vi "letterbox_resize_cubic_planar.vi"(7 "pad Color":u32(colorbox)=7500402, 8 "error in (no error)":errorcluster, 9 "target_h":i32=1024, 10 "target_w":i32=1024, 11 "image in":T1) -> (0 "error out":errorcluster, 1 "out_top":i32, 2 "out_left":i32, 3 "image out":T1, 4 "out_scale":sgl)   [LabVIEW 2017, in "Image Processing Library.lvlib"]
uses:
  Image Processing Library.lvlib
  <vilib>/picture/picture.llb/imagedata.ctl
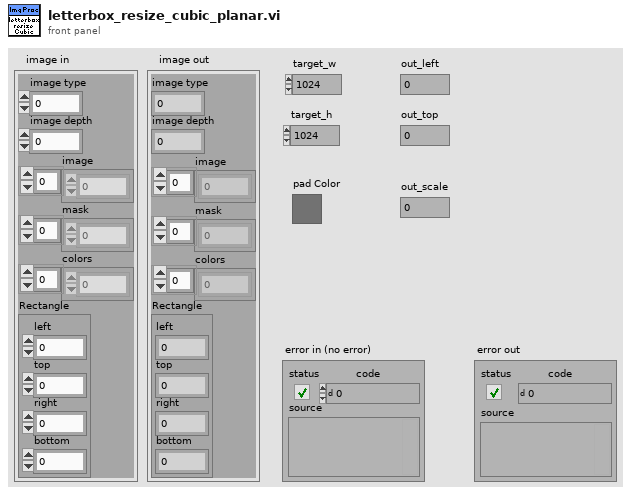
[diagram p1: front panel]
types:
  T1 = typedef "imagedata.ctl" = cluster{"image type":i32, "image depth":i32, "image":u8[], "mask":u8[], "colors":u32[], "Rectangle":cluster{"left":i16, "top":i16, "right":i16, "bottom":i16}}
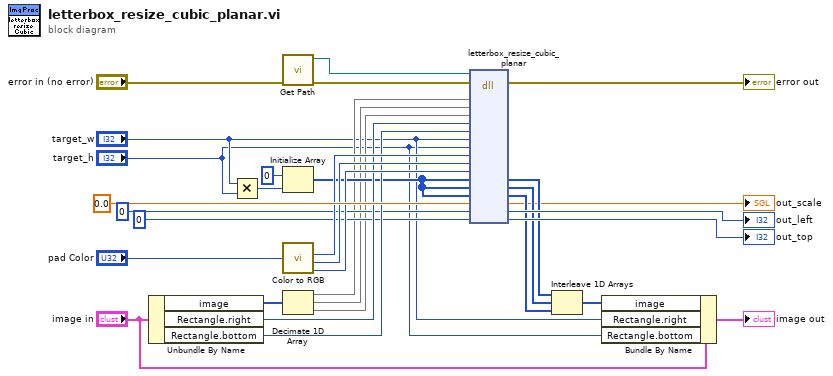
[diagram p0: block diagram]
diagram:
  n1 = Unbundle By Name("image in") -> ("image"=w13:u8[], "Rectangle.right"=w20:i16, "Rectangle.bottom"=w19:i16)
  n2 = Multiply(x="target_w", y="target_h") -> (x*y=w16:i32)
  n3 = call "Get Path.vi"("error in (no error)"="error in (no error)") -> ("error out"=w30:errorcluster, "Library Path"=w29:path)  [unwired: 9 in]
  n4 = Initialize Array(u8 0 ("element"), w16) -> (w14:u8[])
  n5 = call <vilib>:"Color to RGB.vi"("Color"="pad Color") -> ("R"=w25:u8, "G"=w24:u8, "B"=w23:u8)  [unwired: 1 out]
  n6 = Decimate 1D Array(w13) -> (w12:u8[], w11:u8[], w10:u8[])
  n7 = dll-call lib="C:/Users/IvanLis-Win10/Desktop/LabVIEW/Coin Detector/Project_2018/image_processing/windows_x64/image_processing.dll" fn="letterbox_resize_cubic_planar"(path in=w29, error in=w30, "in_r"=w12, "in_g"=w11, "in_b"=w10, "orig_w"=w20, "orig_h"=w19, "target_w"="target_w", "target_h"="target_h", "pad_r"=w25, "pad_g"=w24, "pad_b"=w23, "out_r"=w14, "out_g"=w14, "out_b"=w14, "out_scale"=sgl 0.0, "out_left"=0, "out_top"=0) -> (error out=→"error out":errorcluster, "out_r"=w9:u8[], "out_g"=w8:u8[], "out_b"=w7:u8[], "out_scale"=→"out_scale":sgl, "out_left"=→"out_left":i32, "out_top"=→"out_top":i32)  [unwired: 12 in, 1 out]
  n8 = Interleave 1D Arrays(w9, w8, w7) -> (w6:u8[])
  n9 = Bundle By Name(cluster="image in", "image"=w6, "Rectangle.right"="target_w", "Rectangle.bottom"="target_h") -> (→"image out":T1)
